vi "Test Serializer.Text.vi"(8 "error in (no error)":errorcluster) -> (0 "error out":errorcluster)   [LabVIEW 2013]
uses:
  source/Serializer.PlainText/Serializer.PlainText.lvclass
  <vilib>/addons/_JKI Toolkits/Caraya/classes/Assert/Assert Equal Value and Type_Variant.vi
  <vilib>/addons/_JKI Toolkits/Caraya/classes/Assert/Assert Equal Value_Variant.vi
  <vilib>/addons/_JKI Toolkits/Caraya/classes/Assert/Assert Almost Equal_Float.vi
  <vilib>/addons/_JKI Toolkits/Caraya/classes/Assert/Assert Not Error.vi
  <vilib>/addons/_JKI Toolkits/Caraya/classes/Assert/Assert.lvclass
  source/Serializer/Serializer.lvclass
  <vilib>/addons/_JKI Toolkits/Caraya/classes/Test/Test.lvclass
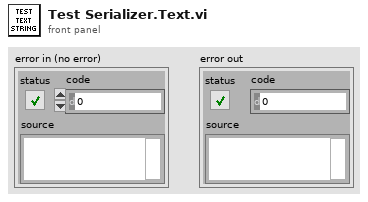
[diagram p1: front panel]
types:
  T1 = cluster{"error":errorcluster, "EnumU16":enum16{"A", "B", "C"}, "Value":dbl, "DBL":dbl[]}
  T2 = cluster{"error":errorcluster, "EnumU16":enum16{"A", "B", "C"}, "Value":dbl}
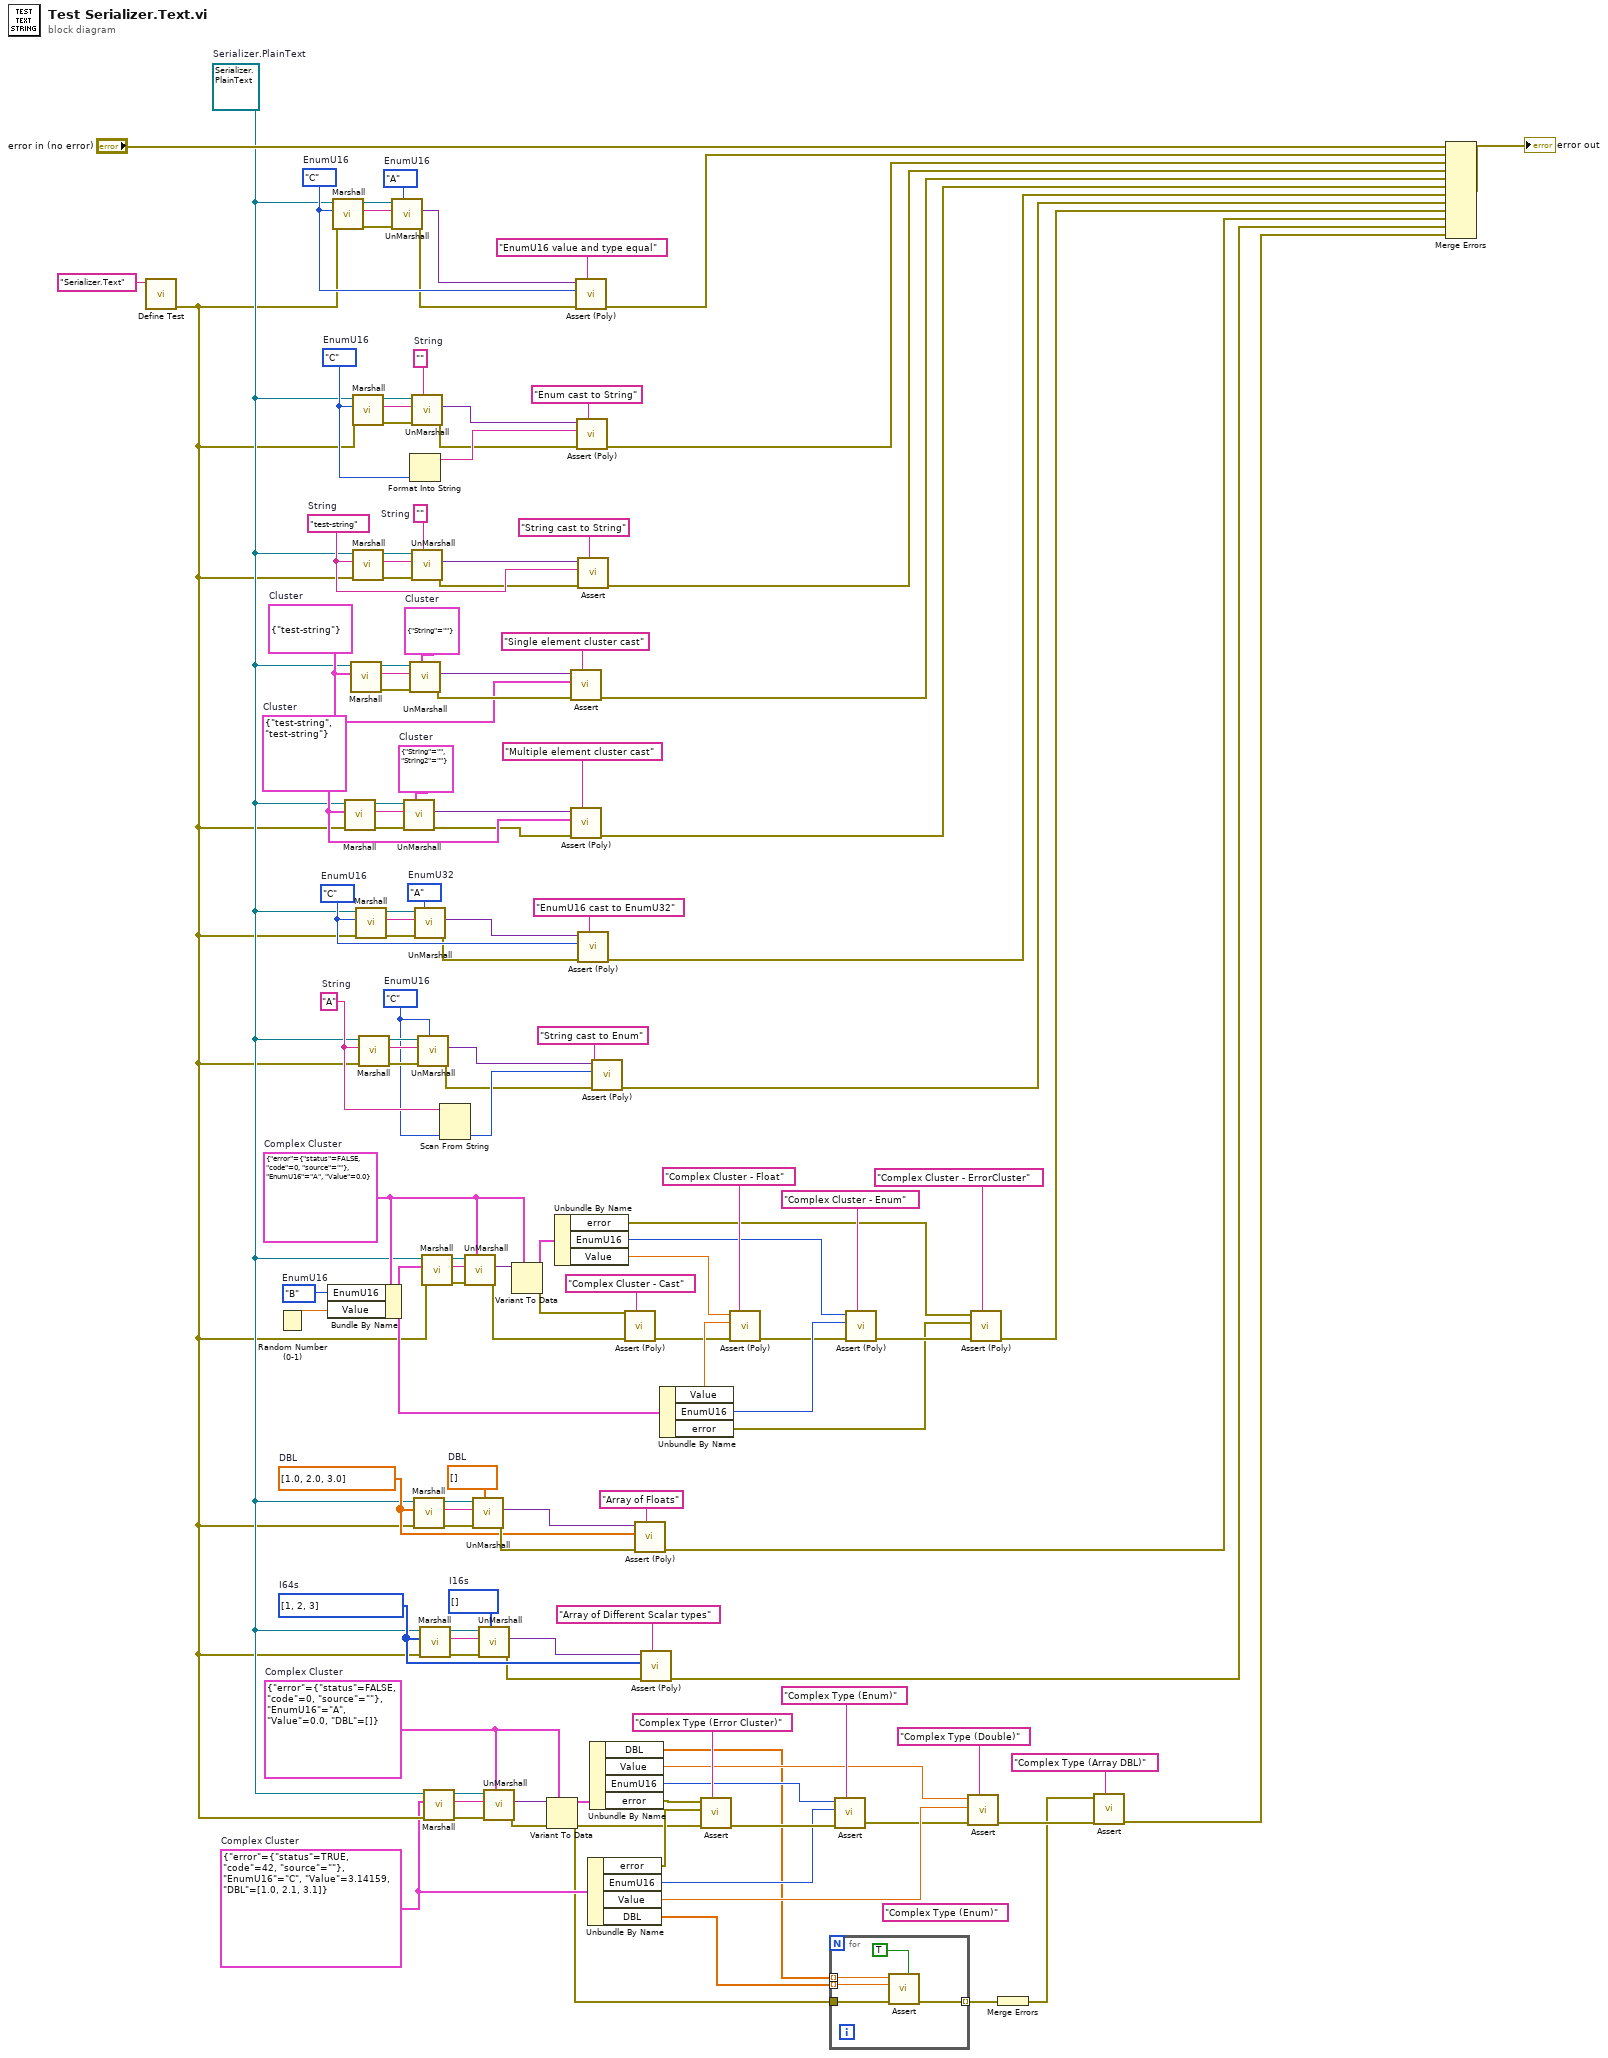
[diagram p0: block diagram]
diagram:
  (unwired) "Complex Type (Enum)" ("Label")
  w21 = T1 {"error"={"status"=TRUE, "code"=42, "source"=""}, "EnumU16"=enum."C", "Value"=3.14159, "DBL"=[1.0, 2.1, 3.1]}  # Complex Cluster
  w20 = T1 {"error"={"status"=FALSE, "code"=0, "source"=""}, "EnumU16"=enum."A", "Value"=0.0, "DBL"=[]}  # Complex Cluster
  w38 = i64[] [1, 2, 3]  # I64s
  w37 = i16[] []  # I16s
  w49 = cluster{"String":string, "String2":string} {"String"="", "String2"=""}  # Cluster
  w47 = cluster{"String":string, "String2":string} {"String"="test-string", "String2"="test-string"}  # Cluster
  w53 = cluster{"String":string} {"String"=""}  # Cluster
  w42 = cluster{"String":string} {"String"="test-string"}  # Cluster
  w61 = "test-string"  # String
  w64 = ""  # String
  w26 = refnum<class "Serializer.PlainText.lvclass"> refnum  # Serializer.PlainText
  w67 = dbl[] [1.0, 2.0, 3.0]  # DBL
  w68 = dbl[] []  # DBL
  w101 = enum16{"A", "B", "C"}."B"  # EnumU16
  w91 = T2 {"error"={"status"=FALSE, "code"=0, "source"=""}, "EnumU16"=enum."A", "Value"=0.0}  # Complex Cluster
  w107 = "A"  # String
  w106 = enum16{"A", "B", "C"}."C"  # EnumU16
  w119 = enum32{"A", "B", "C"}."A"  # EnumU32
  w114 = enum16{"A", "B", "C"}."C"  # EnumU16
  w128 = ""  # String
  w117 = enum16{"A", "B", "C"}."C"  # EnumU16
  w137 = enum16{"A", "B", "C"}."A"  # EnumU16
  w139 = enum16{"A", "B", "C"}."C"  # EnumU16
  n1 = call <vilib>:"Define Test.vi"("Label (VI Title)"="Serializer.Text") -> ("error out"=w25:errorcluster)  [unwired: 10 in]
  n2 = Random Number (0-1)() -> (number: 0 to 1=w100:dbl)
  n3 = Bundle By Name(cluster=w91, "EnumU16"=w101, "Value"=w100) -> (w87:T2)
  n4 = call "Marshall.vi"("error in (no error)"=w25, "Variant"=w139, "Serializer in"=w26) -> ("error out"=w96:errorcluster, "String"=w136:string, "Serializer out"=w135:refnum<class "Serializer.PlainText.lvclass">)  [unwired: 6 in]
  n5 = call "Marshall.vi"("error in (no error)"=w25, "Variant"=w47, "Serializer in"=w26) -> ("error out"=w52:errorcluster, "String"=w51:string, "Serializer out"=w50:refnum<class "Serializer.PlainText.lvclass">)  [unwired: 6 in]
  n6 = call "Marshall.vi"("Variant"=w42, "Serializer in"=w26) -> ("error out"=w54:errorcluster, "String"=w55:string, "Serializer out"=w56:refnum<class "Serializer.PlainText.lvclass">)  [unwired: 7 in]
  n7 = call "Marshall.vi"("error in (no error)"=w25, "Variant"=w117, "Serializer in"=w26) -> ("error out"=w125:errorcluster, "String"=w129:string, "Serializer out"=w130:refnum<class "Serializer.PlainText.lvclass">)  [unwired: 6 in]
  n8 = call "Marshall.vi"("error in (no error)"=w25, "Variant"=w61, "Serializer in"=w26) -> ("error out"=w65:errorcluster, "String"=w63:string, "Serializer out"=w62:refnum<class "Serializer.PlainText.lvclass">)  [unwired: 6 in]
  n9 = call "Marshall.vi"("error in (no error)"=w25, "Variant"=w114, "Serializer in"=w26) -> ("error out"=w124:errorcluster, "String"=w122:string, "Serializer out"=w121:refnum<class "Serializer.PlainText.lvclass">)  [unwired: 6 in]
  n10 = call "Marshall.vi"("error in (no error)"=w25, "Variant"=w107, "Serializer in"=w26) -> ("error out"=w112:errorcluster, "String"=w110:string, "Serializer out"=w109:refnum<class "Serializer.PlainText.lvclass">)  [unwired: 6 in]
  n11 = call "UnMarshall.vi"("Type"=w137, "error in (no error)"=w96, "String"=w136, "Serializer in"=w135) -> ("error out"=w95:errorcluster, "Variant"=w138:variant)  [unwired: 5 in, 1 out]
  n12 = call "UnMarshall.vi"("Type"=w49, "error in (no error)"=w52, "String"=w51, "Serializer in"=w50) -> ("error out"=w44:errorcluster, "Variant"=w48:variant)  [unwired: 5 in, 1 out]
  n13 = Format Into String(w117) -> (resulting string=w116:string)  [unwired: 3 in, 1 out]
  n14 = call "UnMarshall.vi"("Type"=w53, "error in (no error)"=w54, "String"=w55, "Serializer in"=w56) -> ("error out"=w43:errorcluster, "Variant"=w41:variant)  [unwired: 5 in, 1 out]
  n15 = call "UnMarshall.vi"("Type"=w128, "error in (no error)"=w125, "String"=w129, "Serializer in"=w130) -> ("error out"=w97:errorcluster, "Variant"=w118:variant)  [unwired: 5 in, 1 out]
  n16 = call "UnMarshall.vi"("Type"=w64, "error in (no error)"=w65, "String"=w63, "Serializer in"=w62) -> ("error out"=w59:errorcluster, "Variant"=w60:variant)  [unwired: 5 in, 1 out]
  n17 = call "Marshall.vi"("error in (no error)"=w25, "Variant"=w67, "Serializer in"=w26) -> ("error out"=w69:errorcluster, "String"=w71:string, "Serializer out"=w72:refnum<class "Serializer.PlainText.lvclass">)  [unwired: 6 in]
  n18 = call "UnMarshall.vi"("Type"=w119, "error in (no error)"=w124, "String"=w122, "Serializer in"=w121) -> ("error out"=w98:errorcluster, "Variant"=w115:variant)  [unwired: 5 in, 1 out]
  n19 = call "UnMarshall.vi"("Type"=w106, "error in (no error)"=w112, "String"=w110, "Serializer in"=w109) -> ("error out"=w99:errorcluster, "Variant"=w113:variant)  [unwired: 5 in, 1 out]
  n20 = call "Marshall.vi"("error in (no error)"=w25, "Variant"=w38, "Serializer in"=w26) -> ("error out"=w36:errorcluster, "String"=w34:string, "Serializer out"=w33:refnum<class "Serializer.PlainText.lvclass">)  [unwired: 6 in]
  n21 = call "Marshall.vi"("error in (no error)"=w25, "Variant"=w87, "Serializer in"=w26) -> ("error out"=w94:errorcluster, "String"=w103:string, "Serializer out"=w104:refnum<class "Serializer.PlainText.lvclass">)  [unwired: 6 in]
  n22 = call "Marshall.vi"("error in (no error)"=w25, "Variant"=w21, "Serializer in"=w26) -> ("error out"=w29:errorcluster, "String"=w28:string, "Serializer out"=w27:refnum<class "Serializer.PlainText.lvclass">)  [unwired: 6 in]
  n23 = Scan From String(input string=w107, default 1=w106) -> (output 1=w105:enum16{"A", "B", "C"})  [unwired: 3 in, 3 out]
  n24 = call "UnMarshall.vi"("Type"=w91, "error in (no error)"=w94, "String"=w103, "Serializer in"=w104) -> ("error out"=w93:errorcluster, "Variant"=w92:variant)  [unwired: 5 in, 1 out]
  n25 = call "UnMarshall.vi"("Type"=w68, "error in (no error)"=w69, "String"=w71, "Serializer in"=w72) -> ("error out"=w74:errorcluster, "Variant"=w73:variant)  [unwired: 5 in, 1 out]
  n26 = call "UnMarshall.vi"("Type"=w37, "error in (no error)"=w36, "String"=w34, "Serializer in"=w33) -> ("error out"=w31:errorcluster, "Variant"=w32:variant)  [unwired: 5 in, 1 out]
  n27 = call "UnMarshall.vi"("Type"=w20, "error in (no error)"=w29, "String"=w28, "Serializer in"=w27) -> ("error out"=w23:errorcluster, "Variant"=w24:variant)  [unwired: 5 in, 1 out]
  n28 = Variant To Data(type=w91, Variant=w92) -> (data=w89:T2, error out=w90:errorcluster)  [unwired: 1 in]
  n29 = Variant To Data(error in=w23, type=w20, Variant=w24) -> (data=w22:T1, error out=w6:errorcluster)
  n30 = Unbundle By Name(w89) -> ("error"=w76:errorcluster, "EnumU16"=w83:enum16{"A", "B", "C"}, "Value"=w88:dbl)
  n31 = call-poly <vilib>:"Assert.vi"("Label"="Single element cluster cast", "error in (no error)"=w43, "Y"=w42, "X"=w41) -> ("error out"=w39:errorcluster)  [unwired: 7 in]
  n32 = call-poly <vilib>:"Assert (Poly).vi"("Label"="Multiple element cluster cast", "error in (no error)"=w44, "Y"=w47, "X"=w48) -> ("error out"=w45:errorcluster)  [unwired: 7 in]
  n33 = call-poly <vilib>:"Assert (Poly).vi"("Label"="EnumU16 value and type equal", "error in (no error)"=w95, "Y"=w139, "X"=w138) -> ("error out"=w131:errorcluster)  [unwired: 7 in]
  n34 = call-poly <vilib>:"Assert (Poly).vi"("Label"="Enum cast to String", "error in (no error)"=w97, "Y"=w116, "X"=w118) -> ("error out"=w126:errorcluster)  [unwired: 7 in]
  n35 = call-poly <vilib>:"Assert.vi"("Label"="String cast to String", "error in (no error)"=w59, "Y"=w61, "X"=w60) -> ("error out"=w57:errorcluster)  [unwired: 7 in]
  n36 = call-poly <vilib>:"Assert (Poly).vi"("Label"="EnumU16 cast to EnumU32", "error in (no error)"=w98, "Y"=w114, "X"=w115) -> ("error out"=w120:errorcluster)  [unwired: 7 in]
  n37 = Unbundle By Name(w21) -> ("error"=w18:errorcluster, "EnumU16"=w14:enum16{"A", "B", "C"}, "Value"=w11:dbl, "DBL"=w8:dbl[])
  n38 = Unbundle By Name(w22) -> ("DBL"=w7:dbl[], "Value"=w12:dbl, "EnumU16"=w13:enum16{"A", "B", "C"}, "error"=w19:errorcluster)
  n39 = call-poly <vilib>:"Assert (Poly).vi"("Label"="String cast to Enum", "error in (no error)"=w99, "Y"=w105, "X"=w113) -> ("error out"=w108:errorcluster)  [unwired: 7 in]
  n40 = call-poly <vilib>:"Assert (Poly).vi"("Label"="Complex Cluster - Cast", "error in (no error)"=w93, "Not Error?"=w90) -> ("error out"=w85:errorcluster)  [unwired: 8 in]
  n41 = call-poly <vilib>:"Assert (Poly).vi"("Label"="Array of Floats", "error in (no error)"=w74, "Y"=w67, "X"=w73) -> ("error out"=w66:errorcluster)  [unwired: 7 in]
  n42 = call-poly <vilib>:"Assert (Poly).vi"("Label"="Array of Different Scalar types", "error in (no error)"=w31, "Y"=w38, "X"=w32) -> ("error out"=w30:errorcluster)  [unwired: 7 in]
  n43 = Unbundle By Name(w87) -> ("Value"=w86:dbl, "EnumU16"=w81:enum16{"A", "B", "C"}, "error"=w75:errorcluster)
  n44 = call-poly <vilib>:"Assert.vi"("Label"="Complex Type (Error Cluster)", "error in (no error)"=w6, "Y"=w18, "X"=w19) -> ("error out"=w15:errorcluster)  [unwired: 7 in]
  n45 = call-poly <vilib>:"Assert (Poly).vi"("Label"="Complex Cluster - Float", "error in (no error)"=w85, "Y"=w86, "X"=w88) -> ("error out"=w80:errorcluster)  [unwired: 7 in]
  n46 = for {
    tunnel: w8 -> [w145] mode=indexing
    tunnel: w7 -> [w144] mode=indexing
    tunnel: w6 -> [w143]
    tunnel: [w141] -> w3 mode=indexing
    n47 = call-poly <vilib>:"Assert.vi"("Assert Only? (F)"=TRUE, "error in (no error)"=w143, "Y"=w145, "X"=w144) -> ("error out"=w141:errorcluster)  [unwired: 7 in]
  }
  n48 = call-poly <vilib>:"Assert.vi"("Label"="Complex Type (Enum)", "error in (no error)"=w15, "Y"=w14, "X"=w13) -> ("error out"=w10:errorcluster)  [unwired: 7 in]
  n49 = call-poly <vilib>:"Assert (Poly).vi"("Label"="Complex Cluster - Enum", "error in (no error)"=w80, "Y"=w81, "X"=w83) -> ("error out"=w79:errorcluster)  [unwired: 7 in]
  n50 = call-poly <vilib>:"Assert.vi"("Label"="Complex Type (Double)", "error in (no error)"=w10, "Y"=w11, "X"=w12) -> ("error out"=w5:errorcluster)  [unwired: 7 in]
  n51 = call-poly <vilib>:"Assert (Poly).vi"("Label"="Complex Cluster - ErrorCluster", "error in (no error)"=w79, "Y"=w75, "X"=w76) -> ("error out"=w78:errorcluster)  [unwired: 7 in]
  n52 = Merge Errors(w3) -> (w2:errorcluster)
  n53 = call-poly <vilib>:"Assert.vi"("Label"="Complex Type (Array DBL)", "error in (no error)"=w5, "Not Error?"=w2) -> ("error out"=w1:errorcluster)  [unwired: 8 in]
  n54 = Merge Errors("error in (no error)", w131, w126, w57, w39, w45, w120, w108, w78, w66, w30, w1) -> (→"error out":errorcluster)
